vi "Day Rollup.vi"(8 "error in":errorcluster, 9 "Now":timestamp, 10 "Day Entries":T1, 11 "Project Store in":refnum<class "Project Store.lvclass">) -> (0 "error out":errorcluster, 1 "Row Copy Text":string[](array[string]), 2 "Rollup Rows":string[][](array[string]), 3 "Project Store out":refnum<class "Project Store.lvclass">, 5 "All Copy Text":string)   [LabVIEW 2026]
doc: "Rolls a day's time entries up into one line per task for a timesheet. Entries with the same Project ID and Task ID become one row; rows are in the order of each pair's first Start Time. Hours is the summed duration (End minus Start; a running entry with End Time 0 counts up to Now), rounded to the nearest quarter hour with halves rounded up (7.5 min rounds up), and formatted with exactly two decimals and a period (1.25). A pair that rounds to 0.00 still gets a row. Descriptions are the pair's descriptions in Start Time order joined with \"; \", skipping empty ones and exact repeats. Project and task names come from the Project Store; an ID it does not know is shown as the ID itself. An empty Day Entries gives empty outputs and no error.\n\nInputs: Project Store in; Day Entries; Now; error in.\nOutputs: Project Store out; Rollup Rows (Project, Task, Hours, Descriptions); Row Copy Text (each row's Descriptions, for the clipboard); All Copy Text (every row as Project TAB Task TAB Hours TAB Descriptions, rows joined by CR LF, to paste into a spreadsheet); error out.\n\nGenerated by: Claude"
uses:
  Storage/Project Store/Project Store.lvclass
  Storage/Rows/Time Entry List.ctl
  Storage/Rows/Time Entry.ctl
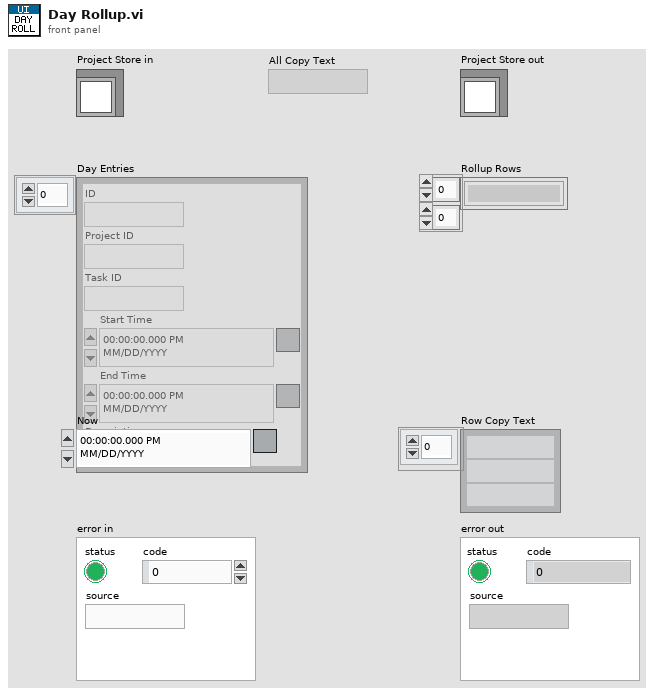
[diagram p1: front panel]
types:
  T1 = typedef "Time Entry List.ctl" = T2[]
  T2 = typedef "Time Entry.ctl" = cluster{"ID":string, "Project ID":string, "Task ID":string, "Start Time":timestamp, "End Time":timestamp, "Description":string}
  T3 = typedef "Project.ctl" = cluster{"ID":string, "Name":string, "Active":bool, "Sort Order":i32}
  T4 = typedef "Task.ctl" = cluster{"ID":string, "Project ID":string, "Name":string, "Active":bool, "Sort Order":i32}
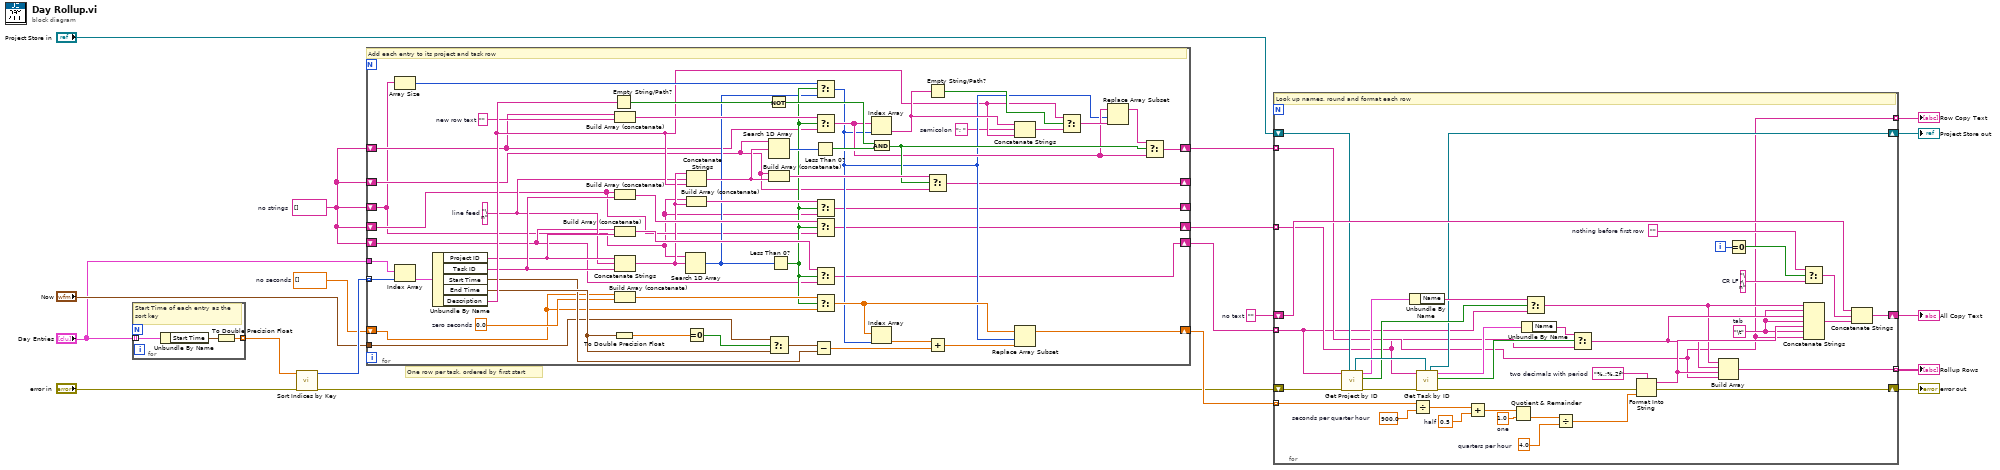
[diagram p0: block diagram]
diagram:
  w12 = ""  # no text
  w11 = dbl[] []  # no seconds
  w10 = string[] []  # no strings
  # "One row per task, ordered by first start"
  n1 = for {
    tunnel: "Day Entries" -> [w20] mode=indexing
    tunnel: [w22] -> w13 mode=indexing
    # "Start Time of each entry as the sort key"
    n2 = Unbundle By Name(w20) -> ("Start Time"=w21:timestamp)
    n3 = To Double Precision Float(number=w21) -> (double precision float=w22:dbl)
  }
  n4 = call "Sort Indices by Key.vi"("error in (no error)"="error in", "Keys"=w13) -> ("error out"=w14:errorcluster, "Sorted Indices"=w15:i32[])  [unwired: 8 in]
  n5 = for {
    tunnel: "Day Entries" -> [w24]
    tunnel: "Now" -> [w25]
    shift-right: [w27] -> _
    shift-left: w10 -> [w26]
    shift-right: [w29] -> w16
    shift-left: w10 -> [w28]
    shift-right: [w31] -> w17
    shift-left: w10 -> [w30]
    shift-right: [w33] -> w18
    shift-left: w11 -> [w32]
    shift-right: [w35] -> w19
    shift-left: w10 -> [w34]
    shift-right: [w37] -> _
    shift-left: w10 -> [w36]
    tunnel: w15 -> [w23] mode=indexing
    w41 = ""  # new row text
    w40 = "; "  # semicolon
    w39 = 0.0  # zero seconds
    w38 = "\n"  # line feed
    # "Add each entry to its project and task row"
    n6 = Array Size(array=w26) -> (size(s)=w55:i32)
    n7 = Index Array(array=w24, index=w23) -> (element=w42:T2)
    n8 = Unbundle By Name(w42) -> ("Project ID"=w43:string, "Task ID"=w44:string, "Start Time"=w45:timestamp, "End Time"=w46:timestamp, "Description"=w47:string)
    n9 = Empty String/Path?(string/path=w47) -> (empty?=w66:bool)
    n10 = To Double Precision Float(number=w46) -> (double precision float=w49:dbl)
    n11 = Build Array (concatenate)(w34, w41) -> (w61:string[])
    n12 = Build Array (concatenate)(w30, w44) -> (w59:string[])
    n13 = Build Array (concatenate)(w28, w43) -> (w58:string[])
    n14 = Concatenate Strings(w43, w38, w44) -> (w48:string)
    n15 = Build Array (concatenate)(w32, w39) -> (w60:dbl[])
    n16 = Search 1D Array(1D array=w26, element=w48) -> (index of element=w53:i32)  [unwired: 1 in]
    n17 = Concatenate Strings(w48, w38, w47) -> (w67:string)
    n18 = Build Array (concatenate)(w26, w48) -> (w57:string[])
    n19 = Equal To 0?(x=w49) -> (x = 0?=w50:bool)
    n20 = Not(x=w66) -> (.not. x?=w70:bool)
    n21 = Search 1D Array(1D array=w36, element=w67) -> (index of element=w68:i32)  [unwired: 1 in]
    n22 = Build Array (concatenate)(w36, w67) -> (w72:string[])
    n23 = Select(t=w25, s=w50, f=w46) -> (s? t:f=w51:timestamp)
    n24 = Less Than 0?(x=w53) -> (x < 0?=w54:bool)
    n25 = Subtract(x=w51, y=w45) -> (x-y=w52:dbl)
    n26 = Less Than 0?(x=w68) -> (x < 0?=w69:bool)
    n27 = Select(t=w55, s=w54, f=w53) -> (s? t:f=w56:i32)
    n28 = Select(t=w61, s=w54, f=w34) -> (s? t:f=w63:string[])
    n29 = Select(t=w57, s=w54, f=w26) -> (s? t:f=w27:string[])
    n30 = Select(t=w59, s=w54, f=w30) -> (s? t:f=w31:string[])
    n31 = Select(t=w58, s=w54, f=w28) -> (s? t:f=w29:string[])
    n32 = Select(t=w60, s=w54, f=w32) -> (s? t:f=w62:dbl[])
    n33 = Index Array(array=w63, index=w56) -> (element=w73:string)
    n34 = And(x=w70, y=w69) -> (x .and. y?=w71:bool)
    n35 = Index Array(array=w62, index=w56) -> (element=w64:dbl)
    n36 = Empty String/Path?(string/path=w73) -> (empty?=w74:bool)
    n37 = Select(t=w72, s=w71, f=w36) -> (s? t:f=w37:string[])
    n38 = Add(x=w64, y=w52) -> (x+y=w65:dbl)
    n39 = Concatenate Strings(w73, w40, w47) -> (w75:string)
    n40 = Replace Array Subset(array=w62, new element=w65, index=w56) -> (w33:dbl[])
    n41 = Select(t=w47, s=w74, f=w75) -> (s? t:f=w76:string)
    n42 = Replace Array Subset(array=w63, new element=w76, index=w56) -> (w77:string[])
    n43 = Select(t=w77, s=w71, f=w63) -> (s? t:f=w35:string[])
  }
  n44 = for {
    shift-right: [w84] -> w5
    shift-left: "Project Store in" -> [w83]
    shift-right: [w88] -> w8
    shift-left: w12 -> [w87]
    tunnel: w16 -> [w79] mode=indexing
    tunnel: w17 -> [w80] mode=indexing
    tunnel: w18 -> [w81] mode=indexing
    tunnel: w19 -> [w82] mode=indexing
    tunnel: [w82] -> w7 mode=indexing
    shift-right: [w86] -> w9
    shift-left: w14 -> [w85]
    tunnel: [w113] -> w6 mode=indexing
    i -> [w78]
    w96 = ""  # nothing before first row
    w95 = "\r\n"  # CR LF
    w94 = "\t"  # tab
    w93 = "%.;%.2f"  # two decimals with period
    w92 = 4.0  # quarters per hour
    w91 = 1.0  # one
    w90 = 0.5  # half
    w89 = 900.0  # seconds per quarter hour
    # "Look up names, round and format each row"
    n45 = call-dynamic "Get Project by ID.vi"("Project Store in"=w83, "error in (no error)"=w85, "ID"=w79) -> ("error out"=w97:errorcluster, "found?"=w98:bool, "Project"=w99:T3, "Project Store out"=w100:refnum<class "Project Store.lvclass">)  [unwired: 5 in]
    n46 = Unbundle By Name(w99) -> ("Name"=w104:string)
    n47 = Divide(x=w81, y=w89) -> (x/y=w108:dbl)
    n48 = call-dynamic "Get Task by ID.vi"("Project Store in"=w100, "error in (no error)"=w97, "ID"=w80) -> ("error out"=w101:errorcluster, "found?"=w102:bool, "Task"=w103:T4, "Project Store out"=w84:refnum<class "Project Store.lvclass">)  [unwired: 5 in]
    n49 = Add(x=w108, y=w90) -> (x+y=w109:dbl)
    n50 = Quotient & Remainder(x=w109, y=w91) -> (floor(x/y)=w110:dbl)  [unwired: 1 out]
    n51 = Unbundle By Name(w103) -> ("Name"=w105:string)
    n52 = Select(t=w104, s=w98, f=w79) -> (s? t:f=w106:string)
    n53 = Divide(x=w110, y=w92) -> (x/y=w111:dbl)
    n54 = Select(t=w105, s=w102, f=w80) -> (s? t:f=w107:string)
    n55 = Format Into String(format string=w93, error in=w101, w111) -> (resulting string=w112:string, error out=w86:errorcluster)  [unwired: 1 in]
    n56 = Build Array(w106, w107, w112, w82) -> (w113:string[])
    n57 = Equal To 0?(x=w78) -> (x = 0?=w115:bool)
    n58 = Select(t=w96, s=w115, f=w95) -> (s? t:f=w116:string)
    n59 = Concatenate Strings(w106, w94, w107, w94, w112, w94, w82) -> (w114:string)
    n60 = Concatenate Strings(w87, w116, w114) -> (w88:string)
  }
  "Project Store out" <- w5
  "Rollup Rows" <- w6
  "Row Copy Text" <- w7
  "All Copy Text" <- w8
  "error out" <- w9
